vi "Create Specific.vi"(7 "Direction":T1, 8 "error in (no error)":errorcluster, 9 "Topic Name":T2, 10 "Blackboard Reference":T3 {"refnum" format="%.0x"}, 11 "CIF_Iceoryx_BB in":refnum<class "CIF_Iceoryx_Chn_I64.lvclass">) -> (0 "error out":errorcluster, 1 "Data Variant":variant, 2 "Writer Reference":T4 {"refnum" format="%.0x"}, 3 "CIF_Iceoryx_BB out":refnum<class "CIF_Iceoryx_Chn_I64.lvclass">, 4 "Cluster or Array String":string)   [LabVIEW 2021, in "CIF_Iceoryx_Chn_I64.lvclass"]
uses:
  CIF_Iceoryx_Chn_I64.lvclass
  <vilib>/CIF Foundation/CIF Iceoryx/Refnum/Typedef/BB Writer Refnum.ctl
  <vilib>/CIF Foundation/CIF Iceoryx/Refnum/Typedef/BB Refnum.ctl
  <vilib>/CIF Foundation/CIF Iceoryx/typedef/Topic Full Names.ctl
  ChannelCommon/typedef/Direction.ctl
  CIF_Iceoryx_Chn_I64.lvclass/CIF_Iceoryx_Chn_I64.ctl
  36e90483-8942-4db4-bc0b-2efc3e994069.vi
  <vilib>/CIF Foundation/CIF Iceoryx/SubVIs/Get Path.vi
  <vilib>/CIF Foundation/CIF Iceoryx/SubVIs/Convert Error.vi
  36e90483-8942-4db4-bc0b-2efc3e994069.vi/f164bb55-fadc-406a-97d8-e3295a396b46.vi
  <vilib>/CIF Foundation/CIF Iceoryx/SubVIs/Add Error.vi
  <vilib>/CIF Foundation/CIF Iceoryx/Refnum/BB from Refnum.vi
  <vilib>/CIF Foundation/CIF Iceoryx/Refnum/BB Writer to Refnum.vi
  <vilib>/Utility/error.llb/Trim Whitespace.vi
  <vilib>/CIF Foundation/CIF Iceoryx/SubVIs/Add Error Core.vi
  <vilib>/CIF Foundation/CIF Utilities/DataTypes/Utilities/Get Element Info of Variant.vi
  <vilib>/CIF Foundation/CIF Iceoryx/SubVIs/Get Type String.vi
  <vilib>/CIF Foundation/CIF Utilities/DataTypes/Utilities/Get JSON Descriptor of Variant.vi
  <vilib>/CIF Foundation/CIF Iceoryx/SubVIs/Convert Error Core.vi
  ChannelCommon/ChannelCommon.lvlib
  <vilib>/CIF Foundation/CIF Iceoryx/Iceoryx.lvlib
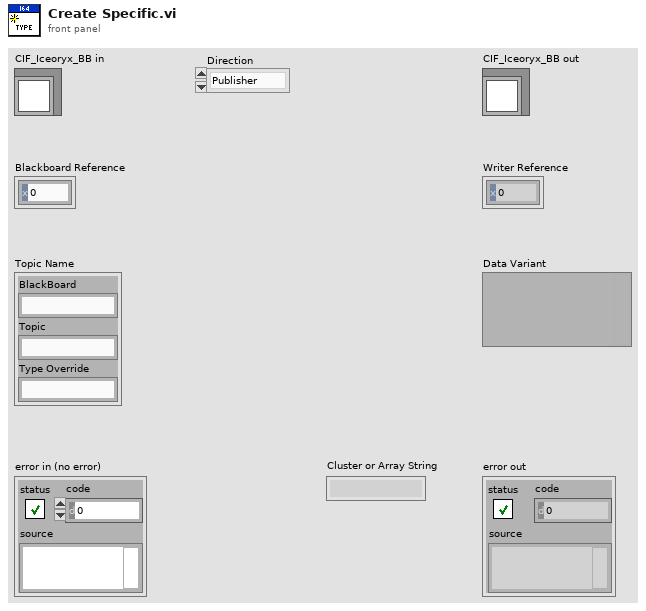
[diagram p1: front panel]
types:
  T1 = typedef "ChannelCommon.lvlib/Direction.ctl" = enum8{"Publisher", "Subscriber"}
  T2 = typedef "Iceoryx.lvlib/Topic Full Names.ctl" = cluster{"BlackBoard":string, "Topic":string, "Type Override":string}
  T3 = typedef "Iceoryx.lvlib/BB Refnum.ctl" = cluster{"refnum":u64, "BB":enum8{"bb"}}
  T4 = typedef "Iceoryx.lvlib/BB Writer Refnum.ctl" = cluster{"refnum":u64, "BB Writer":enum8{"bb_writer"}}
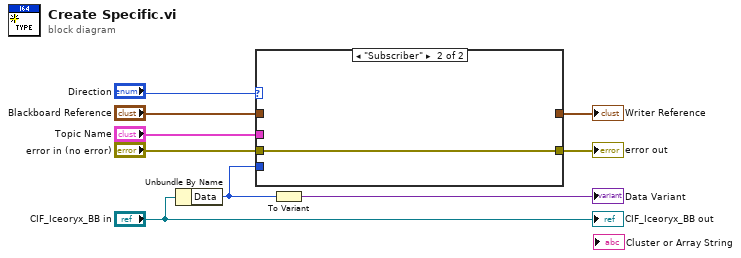
[diagram p0: block diagram]
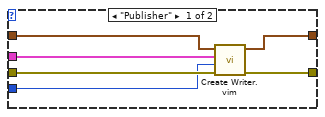
[diagram p2: hidden frame]
diagram:
  n1 = Unbundle By Name("CIF_Iceoryx_BB in") -> ("Data"=w5:i64)
  n2 = case shown="\"Subscriber\"" "Direction" {
    tunnel: "Topic Name" -> [w12 _]
    tunnel: "error in (no error)" -> [w15 w16]
    tunnel: w5 -> [w13 _]
    tunnel: [w14 w16] -> w2
    tunnel: "Blackboard Reference" -> [w11 _]
    tunnel: [w10 _] -> w6
    frame "Publisher" {
      n3 = call "Create Writer.vim"("error in (no error)"=w15, "Data"=w13, "Topic Name"=w12, "BlackBoard Reference"=w11) -> ("error out"=w14:errorcluster, "Writer Reference"=w10:T4)  [unwired: 5 in, 1 out]
    }
    frame "Subscriber" {
    }
  }
  "error out" <- w2
  "Writer Reference" <- w6
  n4 = To Variant(anything=w5) -> (Variant=→"Data Variant":variant)
  "CIF_Iceoryx_BB out" <- "CIF_Iceoryx_BB in"
